vi "Create DIO Panel.vi"(8 "error in (no error)":errorcluster) -> (0 "error out":errorcluster, 3 "Panel Enqueuer":refnum<class "Message Enqueuer.lvclass">)   [LabVIEW 2021, in "Simulator-Channel.lvlib"]
uses:
  Channels/DIO-Channel/Simulator-Channel.lvlib
  <vilib>/ActorFramework/Message Enqueuer/Message Enqueuer.lvclass
  DIO_Panel/DIO_Panel.lvclass
  C:/Program Files/National Instruments/LabVIEW 2021/vi.lib/ActorFramework/Actor/Actor.lvclass
  Channels/DIO-Channel/Private/G_Variables.vi
  <vilib>/ActorFramework/Actor/Actor.lvclass
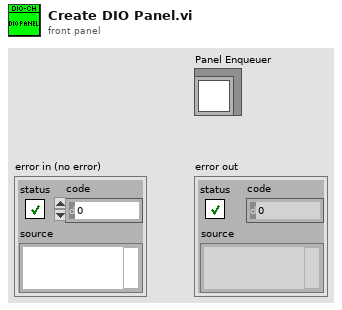
[diagram p1: front panel]
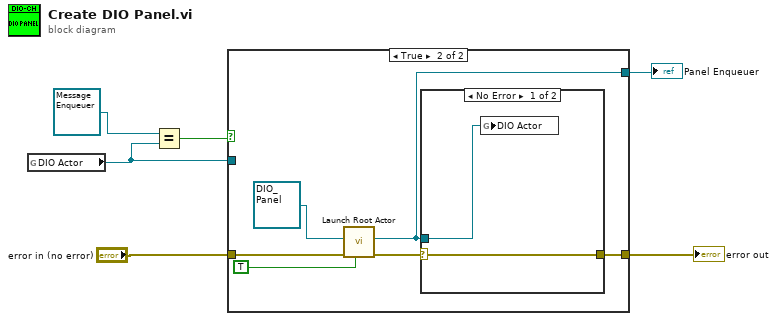
[diagram p0: block diagram]
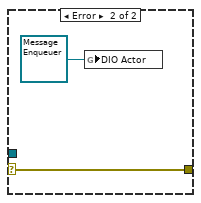
[diagram p3: hidden frame]
diagram:
  n1 = global read "G_Variables.vi" "DIO Actor"() -> (w2:refnum<class "Message Enqueuer.lvclass">)
  n2 = Equal?(x=refnum<class "Message Enqueuer.lvclass"> refnum ("DIO Actor"), y=w2) -> (x = y?=w4:bool)
  n3 = case shown="True" w4 {
    tunnel: "error in (no error)" -> [w7 w14]
    tunnel: [w7 w11] -> w5
    tunnel: [w8 w9] -> w3
    tunnel: w2 -> [w8 _]
    frame False {
    }
    frame True {
      n4 = call <vilib>:"Launch Root Actor.vi"("Open Actor Core front panel? (F)"=TRUE, "error in (no error)"=w14, "Actor"=refnum<class "DIO_Panel.lvclass"> refnum ("Simulator-Channel.lvlib:DIO_Panel.lvlib:UI Template")) -> ("error out"=w10:errorcluster, "Actor's Enqueuer"=w9:refnum<class "Message Enqueuer.lvclass">)  [unwired: 7 in]
      n5 = case shown="No Error" w10 {
        selector: w10 -> [w15 w18]
        tunnel: w9 -> [w16 _]
        tunnel: [w15 w18] -> w11
        frame No Error {
          n6 = global write "G_Variables.vi" "DIO Actor"(w16) -> ()
        }
        frame Error {
          n7 = global write "G_Variables.vi" "DIO Actor"(refnum<class "Message Enqueuer.lvclass"> refnum ("DIO Actor")) -> ()
        }
      }
    }
  }
  "error out" <- w5
  "Panel Enqueuer" <- w3
